vi "VM3 - Variable Data Info.vi"(7 "VC Handle":T3=-1, 8 "error in":errorcluster, 11 "name_spec":string) -> (0 "error out":errorcluster, 1 "stats":T2, 2 "var type":u32, 3 "dup name_spec":string, 4 "has history":bool, 5 "create stats":T1)   [LabVIEW 2021]
doc: "This VI returns information about a variable. Refer to the VI Help for more details.\n\n<b>VC Handle</b> specifies the handle of the variable context. To operate on a global variable, pass -1 to this input. <b>name_spec</b> is the name specifier of the desired variable; usually, it is merely a variable name (see the VI Help for more options).\n\n<b>var type</b> returns the data type code of the variable.\n\n<b>stats</b> returns information about the most recent value of the variable, such as its Writer ID, update time, and update counter.\n\n<b>create stats</b> returns information about the variable creation, such as its Writer ID and create time.\n\n<b>has history</b> returns TRUE if the variable has a history attached.\n\n::: CalcExpress Toolkit :::\nCopyright (c) 2000-2026 Konstantin Shifershteyn. All rights reserved."
uses:
  cetypes.llb/VarMan Variable Context Handle.ctl
  cetypes.llb/VarMan Variable Data Statistics.ctl
  cetypes.llb/VarMan Variable Creation Statistics.ctl
  cetypes.llb/VarMan Error Code.ctl
  cersrc/celveng32.dll
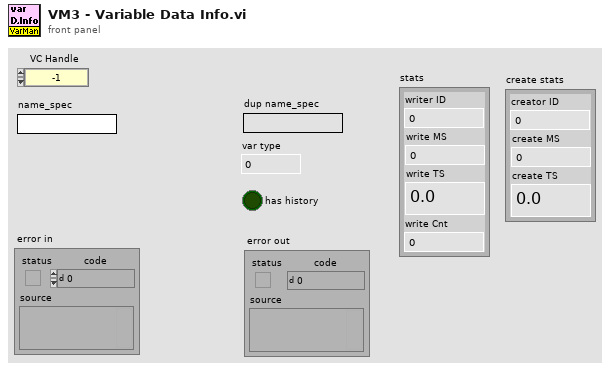
[diagram p1: front panel]
types:
  T1 = typedef "VarMan Variable Creation Statistics.ctl" = cluster{"creator ID":u32, "create MS":u32, "create TS":dbl}
  T2 = typedef "VarMan Variable Data Statistics.ctl" = cluster{"writer ID":u32, "write MS":u32, "write TS":dbl, "write Cnt":u32}
  T3 = typedef "VarMan Variable Context Handle.ctl" = i32
  T4 = typedef "VarMan Error Code.ctl" = u16
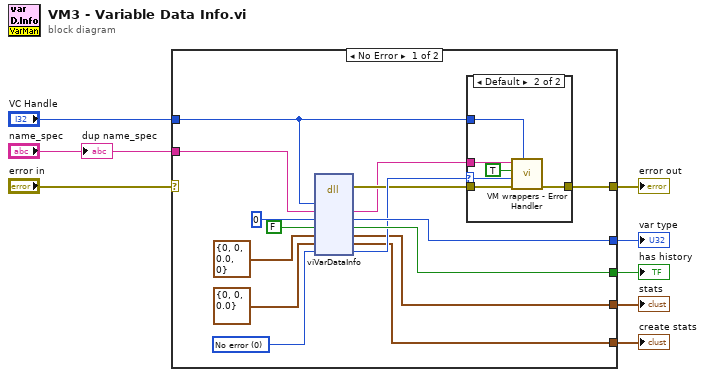
[diagram p0: block diagram]
diagram:
  n1 = case shown="No Error" "error in" {
    selector: "error in" -> [_ w31]
    tunnel: [w23 w31] -> w8
    tunnel: [w22 _] -> w7
    tunnel: "name_spec" -> [w20 _]
    tunnel: "VC Handle" -> [w19 _]
    tunnel: [w18 _] -> w5
    tunnel: [w13 _] -> w2
    tunnel: [w9 _] -> w1
    frame No Error {
      w16 = T4 0 items=["No error", "Invalid variable type", "Variable not found", "Variable already exists", "Invalid context handle", "Input error", "Invalid data format", "No history attached", "History already attached", "Invalid history parameters", "Wrong variable name", "Wrong alias name", "Non-unique alias", "Alias not found", "No alias associated", "Alias already associated", "Wrong context name", "Non-unique context name", "Context name not found", "Invalid parameter", "Generic error", "Memory Full", "Unrecognized LV error", "Unknown error code"] ("VarMan error")
      n2 = dll-call lib="C:/LV Projects/CalcExpress 40 LV2021/vi.lib/addons/CalcExpress/cersrc/celveng*.dll" fn="viVarDataInfo"("vch"=w19, "nspec"=w20, "type"=u32 0, "fHist"=FALSE, "wrStats"=T2 {"writer ID"=0, "write MS"=0, "write TS"=0.0, "write Cnt"=0} ("stats"), "creStats"=T1 {"creator ID"=0, "create MS"=0, "create TS"=0.0} ("create stats"), "errc"=w16) -> (error out=w14:errorcluster, "nspec"=w11:string, "type"=w18:u32, "fHist"=w22:bool, "wrStats"=w13:T2, "creStats"=w9:T1, "errc"=w15:T4)  [unwired: 5 in, 1 out]
      n3 = case shown="Default" w15 {
        selector: w15 -> [_ w25]
        tunnel: w14 -> [w24 w30]
        tunnel: w19 -> [_ w29]
        tunnel: [w24 w28] -> w23
        tunnel: w11 -> [_ w26]
        frame 0 {
        }
        frame Default {
          n4 = call "VM wrappers - Error Handler.vi"("VC Handle"=w29, "error before"=w30, "VarMan error"=w25, "show name spec (F)"=TRUE, "name spec"=w26) -> ("error out"=w28:errorcluster)  [unwired: 5 in, 1 out]
        }
      }
    }
    frame Error {
    }
  }
  "error out" <- w8
  "var type" <- w5
  "has history" <- w7
  "stats" <- w2
  "create stats" <- w1
  "dup name_spec" <- "name_spec"
